vi "Test_C_Frames_To_CIF.vi"() -> ()   [LabVIEW 2021]
uses:
  CANsub_C.lvlib
  C_RX_State.ctl
  api/CANsub_Channel/CANsub_Channel.lvclass
  api/CANsub_API.lvlib
  api/Pcap/CANsub_Pcap_Options.ctl
  api/Pcap/CANsub_Pcap_Results.ctl
panel:
  out "error out":errorcluster
  out "frames decoded":i32
  out "pcap bytes":u8[](array[numeric]) format="%02x"
  out "result":T1
  in  "options":T2={"allow list"=[], "deny list"=[], "TAI minus UTC (s)"=37, "keep TX acks"=FALSE, "little endian"=FALSE}
  in  "max packets":i32
  in  "first":i32
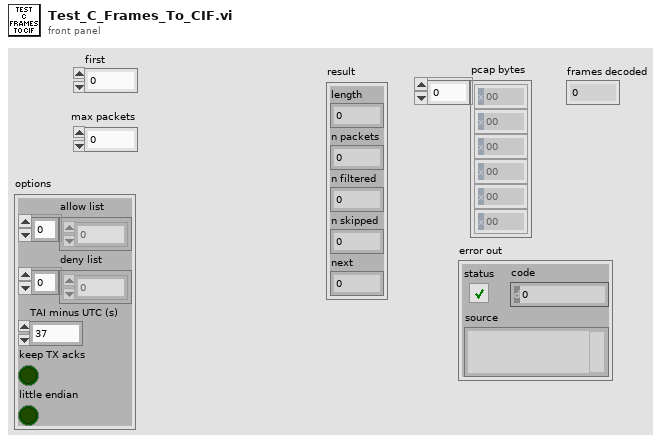
[diagram p1: front panel]
types:
  T1 = typedef "CANsub_API.lvlib/CANsub_Pcap_Results.ctl" = cluster{"length":i32, "n packets":i32, "n filtered":i32, "n skipped":i32, "next":i32}
  T2 = typedef "CANsub_API.lvlib/CANsub_Pcap_Options.ctl" = cluster{"allow list":u32[], "deny list":u32[], "TAI minus UTC (s)":i32, "keep TX acks":bool, "little endian":bool}
  T3 = typedef "CANsub_C.lvlib/C_RX_State.ctl" = cluster{"ws":u8[], "hdlc":u8[], "ping":u8[]}
  T4 = typedef "CANsub_C.lvlib/C_RX_Buffers.ctl" = cluster{"t_dev":dbl[], "ws":u8[], "id":u32[], "flags":u16[], "hdlc":u8[], "dlc":u8[], "data len":u8[], "data":u8[], "ping":u8[]}
  T5 = typedef "CANsub_API.lvlib/CANsub_Frames.ctl" = cluster{"count":i32, "t_dev":dbl[], "id":u32[], "flags":u16[], "dlc":u8[], "data len":u8[], "data":u8[]}
  T6 = typedef "CANsub_C.lvlib/C_Decode_Result.ctl" = cluster{"n frames":i32, "peer close":bool, "ping len":i32, "crc errors":u32, "decode errors":i32}
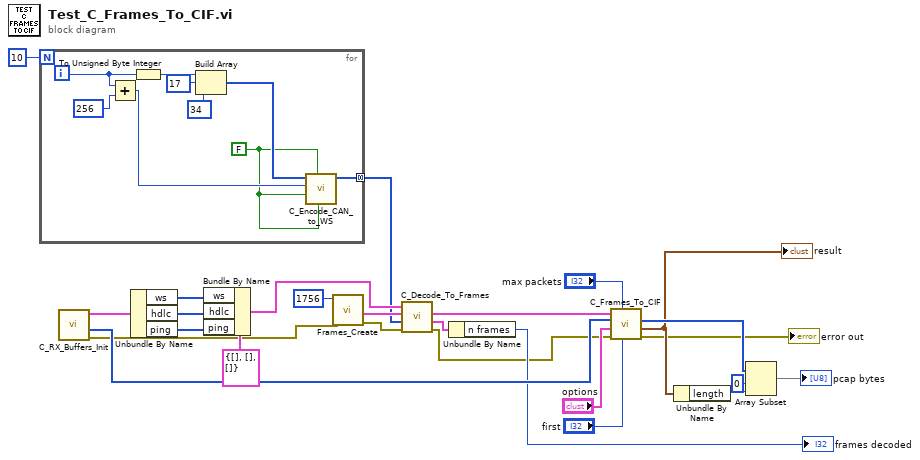
[diagram p0: block diagram]
diagram:
  n1 = for {
    N: 10 -> [_]
    tunnel: [w30] -> w17 mode=concatenating
    i -> [w33]
    w27 = FALSE ("ide")
    n2 = Add(x=w33, y=u32 256) -> (x+y=w29:u32)
    n3 = To Unsigned Byte Integer(number=w33) -> (unsigned 8bit integer=w34:u8)
    n4 = Build Array(w34, u8 17 ("element"), u8 34 ("element")) -> (w28:u8[])
    n5 = call "C_Encode_CAN_to_WS.vi"("brs"=w27, "ide"=w27, "fdf"=w27, "id"=w29, "data"=w28) -> ("ws frame"=w30:u8[])  [unwired: 5 in, 1 out]
  }
  n6 = call "C_RX_Buffers_Init.vi"() -> ("error out"=w2:errorcluster, "pcap"=w14:u8[], "buffers"=w24:T4)  [unwired: 8 in, 1 out]
  n7 = Unbundle By Name(w24) -> ("ws"=w23:u8[], "hdlc"=w22:u8[], "ping"=w21:u8[])
  n8 = Bundle By Name(cluster=T3 {"ws"=[], "hdlc"=[], "ping"=[]} ("C_RX_State"), "ws"=w23, "hdlc"=w22, "ping"=w21) -> (w18:T3)
  n9 = call "Frames_Create.vi"("error in (no error)"=w2, "capacity"=1756) -> ("error out"=w1:errorcluster, "frames"=w19:T5)  [unwired: 8 in]
  n10 = call "C_Decode_To_Frames.vi"("error in (no error)"=w1, "bytes in"=w17, "frames in"=w19, "state in"=w18) -> ("error out"=w4:errorcluster, "result"=w16:T6, "frames out"=w15:T5)  [unwired: 4 in, 1 out]
  n11 = Unbundle By Name(w16) -> ("n frames"=→"frames decoded":i32)
  n12 = call "C_Frames_To_CIF.vi"("first"="first", "max packets"="max packets", "error in (no error)"=w4, "options"="options", "pcap in"=w14, "frames in"=w15) -> ("error out"=→"error out":errorcluster, "result"=w6:T1, "pcap out"=w10:u8[])  [unwired: 2 in, 1 out]
  "result" <- w6
  n13 = Unbundle By Name(w6) -> ("length"=w9:i32)
  n14 = Array Subset(array=w10, index=0, length=w9) -> (→"pcap bytes":u8[])
